vi "Tester.vi"() -> ()   [LabVIEW 2025]
uses:
  94ba14ef-b0cb-4bc0-bfa0-26a289c781ba.vi
  xPanelWrapper.lvlib
panel:
  out "gainLoaded out":i32
  out "offsetLoaded out":i32
  in  "Load Correction Template":bool
  out "offsetMode out":i32 format="%.0x"
  out "gainMode out":i32 format="%.0x"
  out "defectMode out":i32 format="%.0x"
  out "acq fn rtn":i32
  out "height out":i32
  out "width out":i32
  out "serialNumber out":string
  in  "STOP":bool
  out "error out":errorcluster
  out "Image":T1(plugin-control)
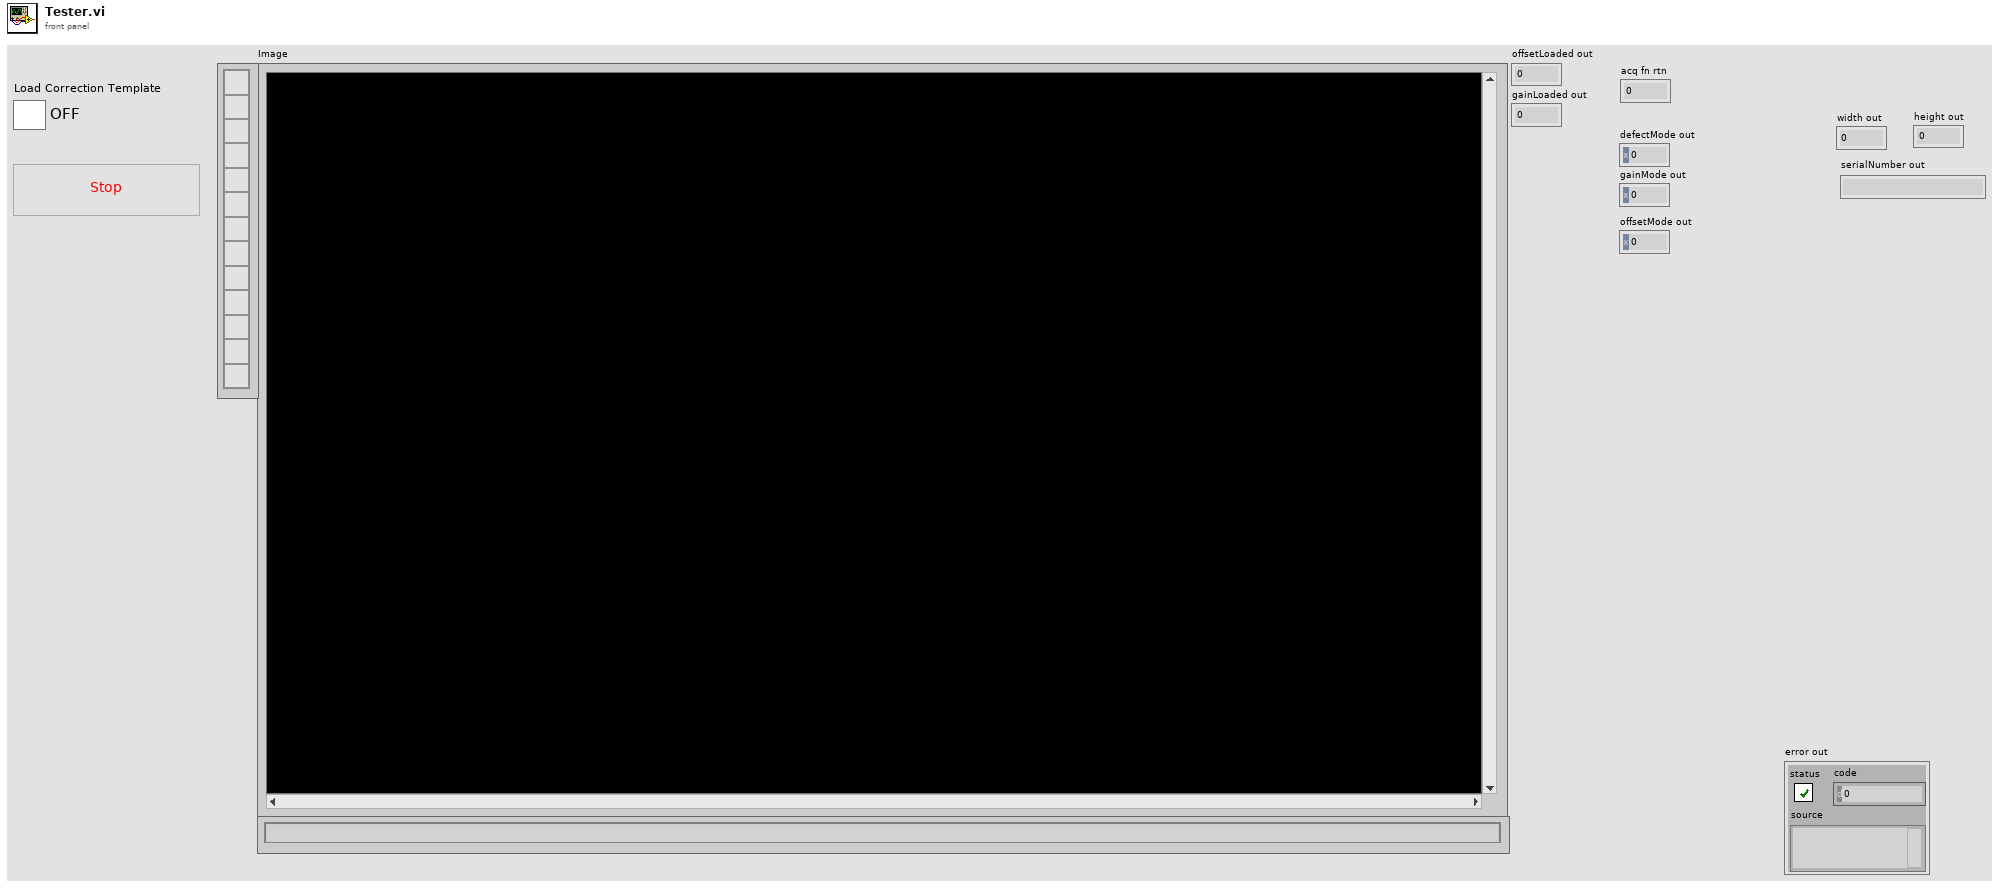
[diagram p1: front panel]
types:
  T1 = typedef "IMAQ Image.ctl" = refnum<image>
  T2 = typedef "Image Type" = u32
  T3 = enum32{"Map Pixel Pointer", "Unmap Pixel Pointer", "Get Pixels Infos"}
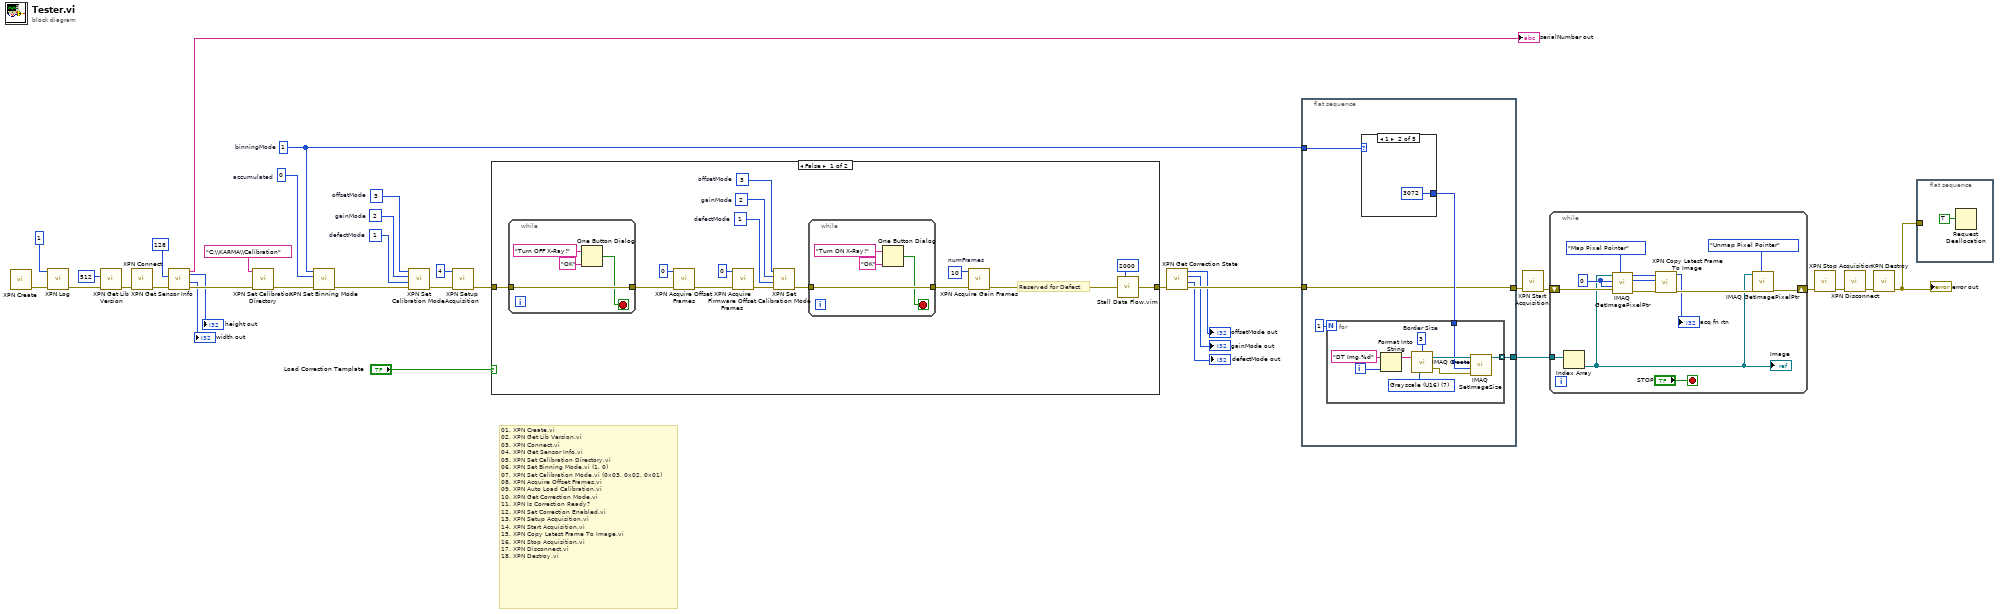
[diagram p0: block diagram]
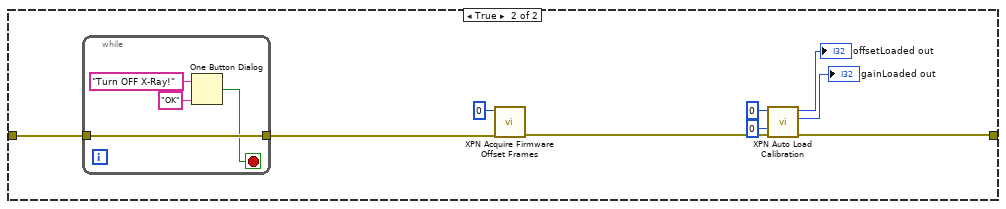
[diagram p2: hidden frame]
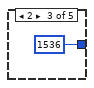
[diagram p4: hidden frame]
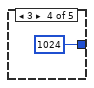
[diagram p5: hidden frame]
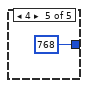
[diagram p6: hidden frame]
diagram:
  w6 = 1  # defectMode
  w7 = 2  # gainMode
  w8 = 3  # offsetMode
  w16 = 1  # binningMode
  w17 = 0  # accumulated
  # "01. XPN Create.vi\n02. XPN Get Lib Version.vi\n03. XPN Connect.vi\n04. XPN Get Sensor Info.vi\n05. XPN Set Calibration Directory.vi\n06. XPN Set Binning Mode.vi (1, 0)\n07. XPN Set Calibration Mode.vi (0x03, 0x02, 0x01)\n08. XPN Acquire Offset Frames.vi\n09. XPN Auto Load Calibration.vi \n10. XPN Get Correction Mode.vi\n11. XPN Is Correction Ready?\n12. XPN Set Correction Enabled.vi\n13. XPN Setup Acquisition.vi\n14. XPN Start Acquisition.vi\n15. XPN Copy Latest Frame To Image.vi\n16. XPN Stop Acquisition.vi\n17. XPN Disconnect.vi\n18. XPN Destroy.vi"
  n1 = call "XPN Create.vi"() -> ("error out"=w35:errorcluster)  [unwired: 10 in, 1 out]
  n2 = call "XPN Log.vi"("error in (no error)"=w35, "enable"=1) -> ("error out"=w2:errorcluster)  [unwired: 8 in, 1 out]
  n3 = call "XPN Get Lib Version.vi"("error in (no error)"=w2, "bufferSize"=512) -> ("error out"=w34:errorcluster)  [unwired: 7 in, 2 out]
  n4 = call "XPN Connect.vi"("error in (no error)"=w34) -> ("error out"=w33:errorcluster)  [unwired: 9 in, 1 out]
  n5 = call "XPN Get Sensor Info.vi"("error in (no error)"=w33, "snSize"=128) -> ("error out"=w31:errorcluster, "width out"=→"width out":i32, "serialNumber out"=→"serialNumber out":string, "height out"=→"height out":i32)  [unwired: 5 in, 1 out]
  n6 = call "XPN Set Calibration Directory.vi"("error in (no error)"=w31, "dirPath"="C:\\KARMA\\Calibration") -> ("error out"=w22:errorcluster)  [unwired: 8 in, 1 out]
  n7 = call "XPN Set Binning Mode.vi"("error in (no error)"=w22, "accumulated"=w17, "binningMode"=w16) -> ("error out"=w10:errorcluster)  [unwired: 7 in, 1 out]
  n8 = call "XPN Set Calibration Mode.vi"("error in (no error)"=w10, "defectMode"=w6, "gainMode"=w7, "offsetMode"=w8) -> ("error out"=w4:errorcluster)  [unwired: 6 in, 1 out]
  n9 = call "XPN Setup Acquisition.vi"("error in (no error)"=w4, "ringBuffCount"=4) -> ("error out"=w3:errorcluster)  [unwired: 8 in, 1 out]
  n10 = case shown="False" "Load Correction Template" {
    tunnel: [w46 w63] -> w11
    tunnel: w3 -> [w44 w64]
    frame False {
      w40 = 1  # defectMode
      w39 = 2  # gainMode
      w38 = 3  # offsetMode
      w47 = 10  # numFrames
      # "Reserved for Defect"
      n11 = while {
        tunnel: w44 -> [w54]
        tunnel: [w54] -> w45
        stop <- w51 stop-if-true
        n12 = One Button Dialog(message="Turn OFF X-Ray!", button name ("OK")="OK") -> (true=w51:bool)
      }
      n13 = call "XPN Acquire Offset Frames.vi"("error in (no error)"=w45, "numFrames"=0) -> ("error out"=w42:errorcluster)  [unwired: 8 in, 1 out]
      n14 = call "XPN Acquire Firmware Offset Frames.vi"("error in (no error)"=w42, "numFrames"=0) -> ("error out"=w37:errorcluster)  [unwired: 8 in, 1 out]
      n15 = call "XPN Set Calibration Mode.vi"("error in (no error)"=w37, "defectMode"=w40, "gainMode"=w39, "offsetMode"=w38) -> ("error out"=w36:errorcluster)  [unwired: 6 in, 1 out]
      n16 = while {
        tunnel: w36 -> [w58]
        tunnel: [w58] -> w50
        stop <- w55 stop-if-true
        n17 = One Button Dialog(message="Turn ON X-Ray!", button name ("OK")="OK") -> (true=w55:bool)
      }
      n18 = call "XPN Acquire Gain Frames.vi"("error in (no error)"=w50, "numFrames"=w47) -> ("error out"=w49:errorcluster)  [unwired: 8 in, 1 out]
      n19 = call "Stall Data Flow.vim"("value in"=w49, "milliseconds to wait"=u32 2000) -> ("value out"=w46:errorcluster)  [unwired: 1 out]
    }
    frame True {
      n20 = while {
        tunnel: w64 -> [w71]
        tunnel: [w71] -> w66
        stop <- w68 stop-if-true
        n21 = One Button Dialog(message="Turn OFF X-Ray!", button name ("OK")="OK") -> (true=w68:bool)
      }
      n22 = call "XPN Acquire Firmware Offset Frames.vi"("error in (no error)"=w66, "numFrames"=0) -> ("error out"=w65:errorcluster)  [unwired: 8 in, 1 out]
      n23 = call "XPN Auto Load Calibration.vi"("error in (no error)"=w65, "gainLoaded"=0, "offsetLoaded"=0) -> ("error out"=w63:errorcluster, "gainLoaded out"=→"gainLoaded out":i32, "offsetLoaded out"=→"offsetLoaded out":i32)  [unwired: 5 in, 1 out]
    }
  }
  n24 = call "XPN Get Correction State.vi"("error in (no error)"=w11) -> ("error out"=w21:errorcluster, "defectMode out"=→"defectMode out":i32, "gainMode out"=→"gainMode out":i32, "offsetMode out"=→"offsetMode out":i32)  [unwired: 6 in, 1 out]
  n25 = flat-sequence {
    tunnel: w21 -> [w72]
    tunnel: [w72] -> w15
    tunnel: [w75] -> w13
    tunnel: w16 -> [w73]
    frame #0 {
      n26 = case shown="1" w73 {
        tunnel: [_ 3072 ("X Resolution") 1536 ("X Resolution") 1024 ("X Resolution") 768 ("X Resolution")] -> w74
        frame 0, Default {
        }
        frame 1 {
        }
        frame 2 {
        }
        frame 3 {
        }
        frame 4 {
        }
      }
      n27 = for {
        N: 1 -> [_]
        tunnel: [w86] -> w75 mode=indexing
        tunnel: w74 -> [w81]
        i -> [w82]
        w85 = 3  # Border Size
        w88 = T2 7 items=["Grayscale (U8)", "Grayscale (I16)", "Grayscale (SGL)", "Complex (CSG)", "RGB (U32)", "HSL (U32)", "RGB (U64)", "Grayscale (U16)"] ("Image Type")
        n28 = Format Into String(initial string="DT Img.%d" ("Image Name"), w82) -> (resulting string=w83:string)  [unwired: 2 in, 1 out]
        n29 = call "IMAQ Create"("Border Size"=w85, "Image Name"=w83, "Image Type"=w88) -> ("New Image"=w87:T1, "error out"=w84:errorcluster)  [unwired: 2 in]
        n30 = call "IMAQ SetImageSize"("error in (no error)"=w84, "Y Resolution"=w81, "X Resolution"=w81, "Image"=w87) -> ("Image Out"=w86:T1)  [unwired: 1 in, 1 out]
      }
    }
  }
  n31 = call "XPN Start Acquisition.vi"("error in (no error)"=w15) -> ("error out"=w14:errorcluster)  [unwired: 9 in, 1 out]
  n32 = while {
    tunnel: w13 -> [w97]
    shift-right: [w94] -> w12
    shift-left: w14 -> [w100]
    stop <- "STOP" stop-if-true
    w101 = 0 ("X Coordinate")
    n33 = Index Array(array=w97) -> (element=w90:T1)  [unwired: 1 in]
    "Image" <- w90
    n34 = call "IMAQ GetImagePixelPtr"("Function"=T3."Map Pixel Pointer", "error in (no error)"=w100, "Y Coordinate"=w101, "X Coordinate"=w101, "Image"=w90) -> ("error out"=w99:errorcluster, "LineWidth(Pixels)"=w98:i32, "Pixel Pointer out"=w92:u64)  [unwired: 1 in, 3 out]
    n35 = call "XPN Copy Latest Frame To Image.vi"("error in (no error)"=w99, "LVLineWidthPixels"=w98, "LVImagePtr"=w92) -> ("error out"=w96:errorcluster, "function return"=→"acq fn rtn":i32)  [unwired: 7 in]
    n36 = call "IMAQ GetImagePixelPtr"("Function"=T3."Unmap Pixel Pointer", "error in (no error)"=w96, "Image"=w90) -> ("error out"=w94:errorcluster)  [unwired: 3 in, 5 out]
  }
  n37 = call "XPN Stop Acquisition.vi"("error in (no error)"=w12) -> ("error out"=w30:errorcluster)  [unwired: 9 in, 1 out]
  n38 = call "XPN Disconnect.vi"("error in (no error)"=w30) -> ("error out"=w29:errorcluster)  [unwired: 9 in, 1 out]
  n39 = call "XPN Destroy.vi"("error in (no error)"=w29) -> ("error out"=w28:errorcluster)  [unwired: 9 in, 1 out]
  "error out" <- w28
  n40 = flat-sequence {
    tunnel: w28 -> [_]
    frame #0 {
      n41 = Request Deallocation(TRUE ("flag")) -> ()
    }
  }
